vi "UTC Offset to Seconds.vi"(11 "UTC Offset String":string) -> (1 "Valid?":bool, 2 "Offset (s)":ext, 3 "UTC Offset":T1=enum."UTC+00:00", 4 "UTC Offset?":bool)   [LabVIEW 2013]
uses:
  UTC Offsets -- enum.ctl
  <vilib>/regexp/Match Regular Expression.xnode
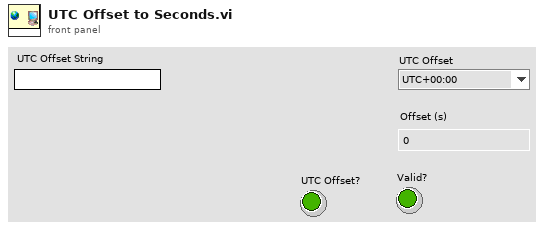
[diagram p1: front panel]
types:
  T1 = typedef "UTC Offsets -- enum.ctl" = enum16{"UTC-12:00", "UTC-11:00", "UTC-10:00", "UTC-09:30", "UTC-09:00", "UTC-08:00", "UTC-07:00", "UTC-06:00", "UTC-05:00", "UTC-04:00", "UTC-03:30", "UTC-03:00", "UTC-02:00", "UTC-01:00", "UTC-00:00", "UTC+00:00", "UTC+01:00", "UTC+02:00", "UTC+03:00", "UTC+03:30", "UTC+04:00", "UTC+04:30", "UTC+05:00", "UTC+05:30", "UTC+05:45", "UTC+06:00", "UTC+06:30", "UTC+07:00", "UTC+08:00", "UTC+08:45", "UTC+09:00", "UTC+09:30", "UTC+10:00", "UTC+10:30", "UTC+11:00", "UTC+12:00", "UTC+12:45", "UTC+13:00", "UTC+14:00"}
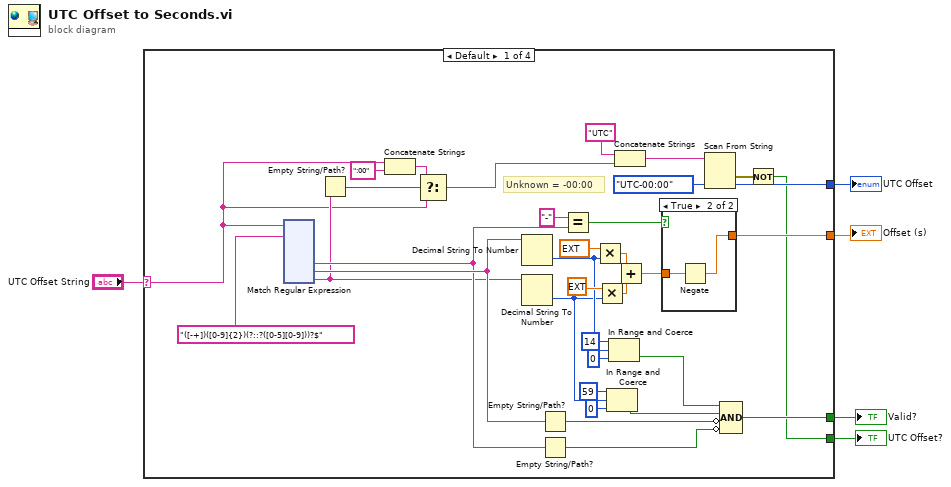
[diagram p0: block diagram]
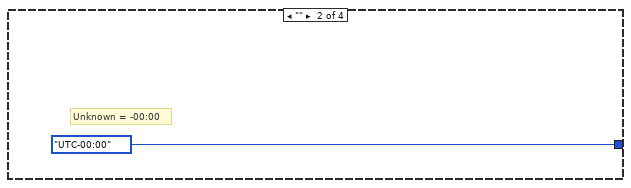
[diagram p3: hidden frame]
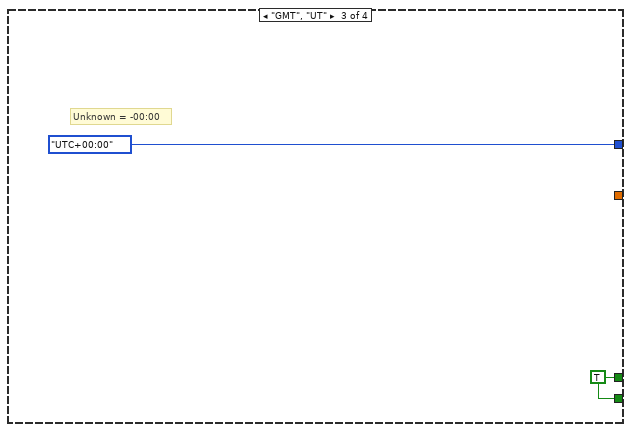
[diagram p4: hidden frame]
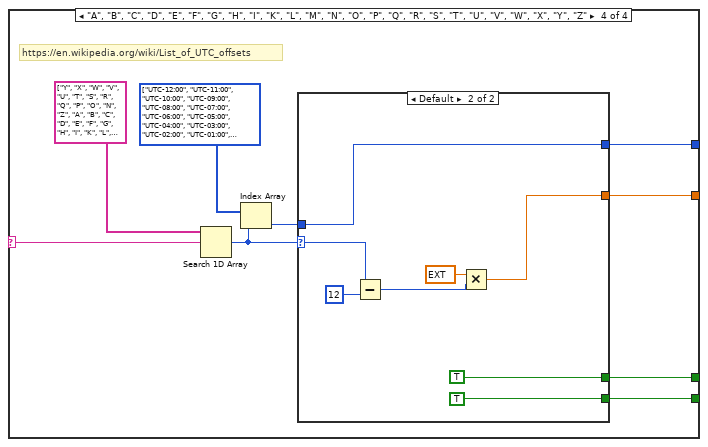
[diagram p5: hidden frame]
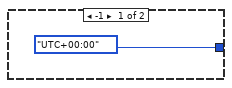
[diagram p6: hidden frame]
diagram:
  n1 = case shown="Default" "UTC Offset String" {
    selector: "UTC Offset String" -> [w9 _ _ w168]
    tunnel: [w38 UTC_Offsets_--_enum."UTC-00:00" ("UTC Time Offset") UTC_Offsets_--_enum."UTC+00:00" ("UTC Time Offset") w172] -> w5
    tunnel: [w28 _ _ w170] -> w4
    tunnel: [w24 _ w162 w171] -> w3
    tunnel: [w6 _ w162 w164] -> w1
    frame Default {
      # "Unknown = -00:00"
      n2 = xnode "Match Regular Expression"("input string"=w9, "regular expression"="([-+])([0-9]{2})(?::?([0-5][0-9]))?$") -> ("submatch 1"=w26:string, "submatch 2"=w27:string, "submatch 3"=w13:string)  [unwired: 4 in, 5 out]
      n3 = Empty String/Path?(string/path=w13) -> (empty?=w12:bool)
      n4 = Concatenate Strings(w9, ":00" ("string")) -> (w11:string)
      n5 = Select(t=w11, s=w12, f=w9) -> (s? t:f=w10:string)
      n6 = Decimal String To Number(string=w27) -> (number=w23:i32)  [unwired: 2 in, 1 out]
      n7 = Decimal String To Number(string=w13) -> (number=w17:i32)  [unwired: 2 in, 1 out]
      n8 = Empty String/Path?(string/path=w27) -> (empty?=w25:bool)
      n9 = Empty String/Path?(string/path=w26) -> (empty?=w14:bool)
      n10 = Equal?(x="-" ("y"), y=w26) -> (x = y?=w29:bool)
      n11 = Multiply(x=ext 3600.0, y=w23) -> (x*y=w33:ext)
      n12 = Multiply(x=ext 60.0, y=w17) -> (x*y=w32:ext)
      n13 = In Range and Coerce(upper limit=59, x=w17, lower limit=0) -> (In Range?=w16:bool)  [unwired: 1 out]
      n14 = In Range and Coerce(upper limit=14, x=w23, lower limit=0) -> (In Range?=w20:bool)  [unwired: 1 out]
      n15 = Concatenate Strings("UTC" ("format string"), w10) -> (w37:string)
      n16 = Add(x=w33, y=w32) -> (x+y=w31:ext)
      n17 = case shown="True" w29 {
        tunnel: w31 -> [w158 w160]
        tunnel: [w158 w159] -> w28
        frame False {
        }
        frame True {
          n18 = Negate(x=w160) -> (-x=w159:ext)
        }
      }
      n19 = Scan From String(input string=w37, default 1=UTC_Offsets_--_enum."UTC-00:00" ("UTC Time Offset")) -> (error out=w7:errorcluster, output 1=w38:T1)  [unwired: 3 in, 2 out]
      n20 = Compound Arithmetic op=AND(w20, w16, invert w25, invert w14) -> (w24:bool)
      n21 = Not(x=w7) -> (.not. x?=w6:bool)
    }
    frame "" {
      # "Unknown = -00:00"
    }
    frame "GMT", "UT" {
      w162 = TRUE
      # "Unknown = -00:00"
    }
    frame "A", "B", "C", "D", "E", "F", "G", "H", "I", "K", "L", "M", "N", "O", "P", "Q", "R", "S", "T", "U", "V", "W", "X", "Y", "Z" {
      w167 = T1[] [enum."UTC-12:00", enum."UTC-11:00", enum."UTC-10:00", enum."UTC-09:00", enum."UTC-08:00", enum."UTC-07:00", enum."UTC-06:00", enum."UTC-05:00", enum."UTC-04:00", enum."UTC-03:00", enum."UTC-02:00", enum."UTC-01:00", enum."UTC+00:00", enum."UTC+01:00", enum."UTC+02:00", enum."UTC+03:00", enum."UTC+04:00", enum."UTC+05:00", enum."UTC+06:00", enum."UTC+07:00", enum."UTC+08:00", enum."UTC+09:00", enum."UTC+10:00", enum."UTC+11:00", enum."UTC+12:00"] items=["UTC-12:00", "UTC-11:00", "UTC-10:00", "UTC-09:30", "UTC-09:00", "UTC-08:00", "UTC-07:00", "UTC-06:00", "UTC-05:00", "UTC-04:00", "UTC-03:30", "UTC-03:00", "UTC-02:00", "UTC-01:00", "UTC-00:00", "UTC+00:00", "UTC+01:00", "UTC+02:00", "UTC+03:00", "UTC+03:30", "UTC+04:00", "UTC+04:30", "UTC+05:00", "UTC+05:30", "UTC+05:45", "UTC+06:00", "UTC+06:30", "UTC+07:00", "UTC+08:00", "UTC+08:45", "UTC+09:00", "UTC+09:30", "UTC+10:00", "UTC+10:30", "UTC+11:00", "UTC+12:00", "UTC+12:45", "UTC+13:00", "UTC+14:00"]
      # "https://en.wikipedia.org/wiki/List_of_UTC_offsets"
      n22 = Search 1D Array(1D array=string[] ["Y", "X", "W", "V", "U", "T", "S", "R", "Q", "P", "O", "N", "Z", "A", "B", "C", "D", "E", "F", "G", "H", "I", "K", "L", "M"], element=w168) -> (index of element=w166:i32)  [unwired: 1 in]
      n23 = Index Array(array=w167, index=w166) -> (element=w165:T1)
      n24 = case shown="Default" w166 {
        selector: w166 -> [_ w177]
        tunnel: [UTC_Offsets_--_enum."UTC+00:00" ("UTC Time Offset") w180] -> w172
        tunnel: [_ TRUE] -> w171
        tunnel: [_ w174] -> w170
        tunnel: w165 -> [_ w180]
        tunnel: [_ TRUE] -> w164
        frame -1 {
        }
        frame Default {
          n25 = Subtract(x=w177, y=12) -> (x-y=w175:i32)
          n26 = Multiply(x=ext 3600.0, y=w175) -> (x*y=w174:ext)
        }
      }
    }
  }
  "UTC Offset" <- w5
  "Offset (s)" <- w4
  "Valid?" <- w3
  "UTC Offset?" <- w1
